vi "Set CanReaderCansub GetCANStatus Response.vi"(7 "Streaming? (F)":bool, 8 "error in (no error)":errorcluster, 10 "Message Data":T1, 11 "gRPCid in":T4) -> (0 "error out":errorcluster)   [LabVIEW 2021, in "CanReaderCansub_server.lvlib" / "CanReaderCansub.lvclass"]
uses:
  CanReaderCansub.lvclass
  <vilib>/gRPC/LabVIEW gRPC Library/Shared/grpcId.ctl
  <vilib>/gRPC/gRPC Server and Client Template [2]/Server Template/RPC Messages/Set package_templatemessage.vi/dcc74a39-081a-4bdd-860b-8ed792803c96.vi
  <vilib>/gRPC/gRPC Server and Client Template [2]/Server Template/RPC Messages/Set package_templatemessage.vi/c8cd2a7d-3f0e-47f4-bd6c-d8bf1e02ce4e.vi
  <vilib>/gRPC/LabVIEW gRPC Library/Shared/TranslateGrpcError.vi
  <vilib>/gRPC/LabVIEW gRPC Library/Server API/Server/Get Server DLL Path.vi
  <vilib>/Utility/error.llb/Error Cluster From Error Code.vi
  <vilib>/gRPC/LabVIEW gRPC Library/Server API/Message Requests/Complete Call.vi
  CanReaderCansub.lvclass/CanReaderCansub.ctl
  CanReaderCansub_server.lvlib
  <vilib>/gRPC/LabVIEW gRPC Library/grpc-lvsupport-release.lvlib
  RPC Messages/cif_can_reader_cansub_LastError.ctl
  RPC Messages/cif_can_reader_cansub_CommState.ctl
  RPC Messages/cif_can_reader_cansub_GetCANStatusResponse.ctl
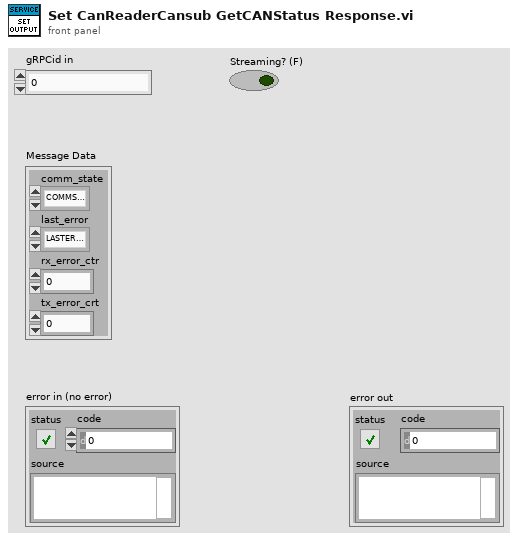
[diagram p1: front panel]
types:
  T1 = typedef "CanReaderCansub_server.lvlib/cif_can_reader_cansub_GetCANStatusResponse.ctl" = cluster{"comm_state":T2, "last_error":T3, "rx_error_ctr":u32, "tx_error_crt":u32}
  T2 = typedef "CanReaderCansub_server.lvlib/cif_can_reader_cansub_CommState.ctl" = enum32{"COMMSTATE_ERROR_ACTIVE", "COMMSTATE_ERROR_PASSIVE", "COMMSTATE_BUS_OFF"}
  T3 = typedef "CanReaderCansub_server.lvlib/cif_can_reader_cansub_LastError.ctl" = enum32{"LASTERROR_NONE", "LASTERROR_STUFF", "LASTERROR_FORM", "LASTERROR_ACK", "LASTERROR_BIT1", "LASTERROR_BIT0", "LASTERROR_CRC", "LASTERROR_UNKNOWN"}
  T4 = typedef "grpc-lvsupport-release.lvlib/grpcId.ctl" = u64
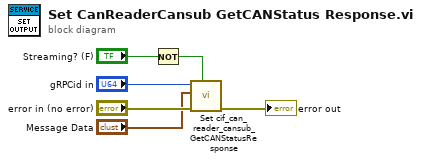
[diagram p0: block diagram]
diagram:
  n1 = Not(x="Streaming? (F)") -> (.not. x?=w1:bool)
  n2 = call "Set cif_can_reader_cansub_GetCANStatusResponse.vi"("Complete Call (T)"=w1, "error in (no error)"="error in (no error)", "package_templatemessage"="Message Data", "gRPCid"="gRPCid in") -> ("error out"=→"error out":errorcluster)  [unwired: 7 in]
